vi "VIH ExtCmd - Check VIHRUN Existence.vi"(8 "error in":errorcluster) -> (0 "error out":errorcluster, 2 "VIHRUN path":path, 3 "Exist":bool, 5 "In LV Folder":bool, 7 "Implemented":bool)   [LabVIEW 2014]
doc: "::: VI Helpeks :::\nCopyright (c) 2000-2026 Konstantin Shifershteyn. All rights reserved."
panel:
  # "VI Helpeks\nCopyright (c) 2012-2026 Konstantin Shifershteyn"
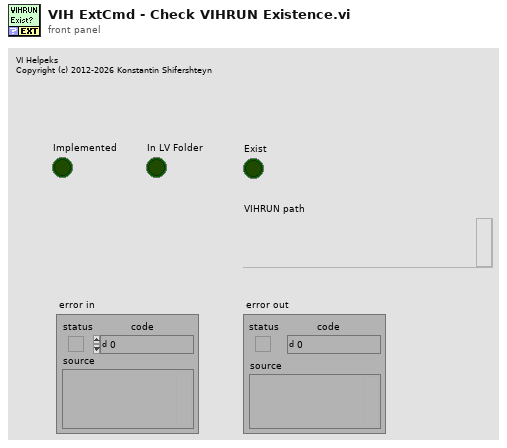
[diagram p1: front panel]
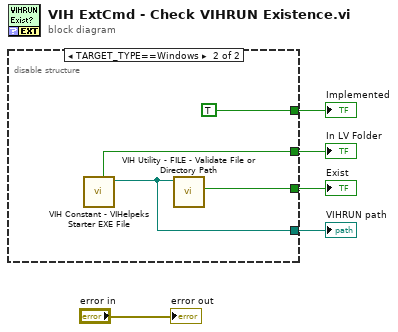
[diagram p0: block diagram]
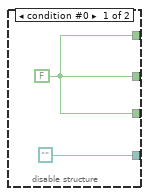
[diagram p2: hidden frame]
diagram:
  n1 = disable-structure shown="TARGET_TYPE==Windows" {
    disable-tunnel: [w6 w11] -> w5
    disable-tunnel: [w6 w10] -> w4
    disable-tunnel: [path "" w9] -> w3
    disable-tunnel: [w6 TRUE] -> w1
    frame condition #0 {
      w6 = FALSE
    }
    frame condition #1 (active) {
      n2 = call "VIH Constant - VIHelpeks Starter EXE File.vi"() -> ("VIHelpeks Starter EXE path"=w9:path, "In LV Folder"=w11:bool)  [unwired: 9 in, 1 out]
      n3 = call "VIH Utility - FILE - Validate File or Directory Path.vi"("Path"=w9) -> ("file"=w10:bool)  [unwired: 6 in, 4 out]
    }
  }
  "Exist" <- w4
  "VIHRUN path" <- w3
  "In LV Folder" <- w5
  "Implemented" <- w1
  "error out" <- "error in"
